vi "add2.vi"(9 "a":dbl, 11 "b":dbl) -> (2 "a*b":dbl)   [LabVIEW 2017]
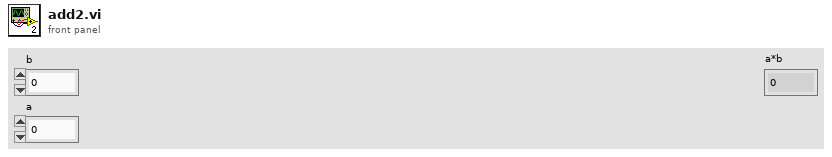
[diagram p1: front panel]
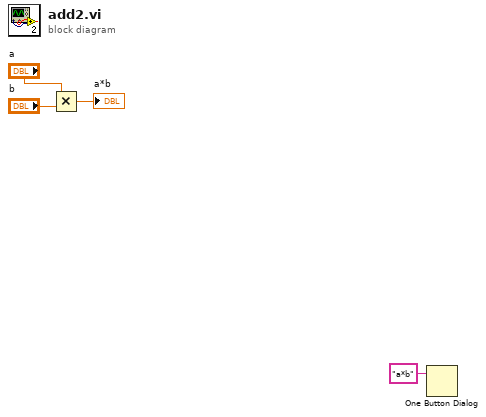
[diagram p0: block diagram]
diagram:
  n1 = Multiply(x="a", y="b") -> (x*y=→"a*b":dbl)
  n2 = One Button Dialog(message="a*b") -> ()  [unwired: 1 in, 1 out]
